vi "Set Logger Enqueuer.vi"(8 "error in":errorcluster, 10 "Logger":refnum<class "Message Enqueuer.lvclass">, 11 "Python Caller in":refnum<class "Python Caller.lvclass">) -> (0 "error out":errorcluster, 3 "Python Caller out":refnum<class "Python Caller.lvclass">)   [LabVIEW 2026, in "Python Caller.lvclass"]
doc: "Set the logger enqueuer for a Logger Client."
uses:
  Python Caller.lvclass
  <vilib>/ActorFramework/Message Enqueuer/Message Enqueuer.lvclass
  Python Caller.lvclass/Python Caller.ctl
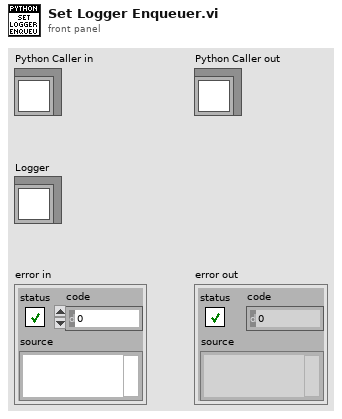
[diagram p1: front panel]
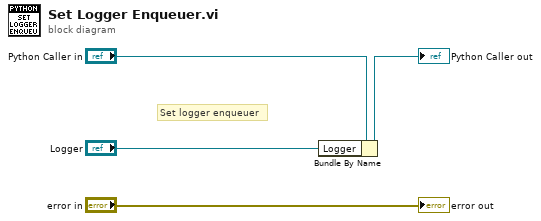
[diagram p0: block diagram]
diagram:
  # "Set logger enqueuer"
  n1 = Bundle By Name(cluster="Python Caller in", "Logger"="Logger") -> (→"Python Caller out":refnum<class "Python Caller.lvclass">)
  "error out" <- "error in"
